vi "ShowWindow Wrapper Template.vi"(0 "hWnd":u64, 5 "nCmdShow":i32=4, 11 "error in":errorcluster) -> (4 "return value":i32, 15 "error out":errorcluster)   [LabVIEW 2020]
doc: "Sets the show state of the window hWnd through user32.dll ShowWindow (stdcall, called in any thread). nCmdShow 4 SW_SHOWNOACTIVATE restores a minimized window without activating it; 9 SW_RESTORE restores and activates; 0 SW_HIDE hides it. When error in carries an error the DLL is not called. Generated by tools\\Build Win32 Wrappers.vi - do not edit by hand, rebuild it."
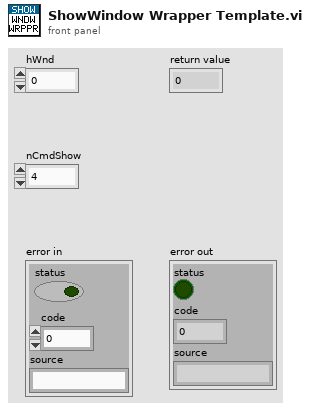
[diagram p1: front panel]
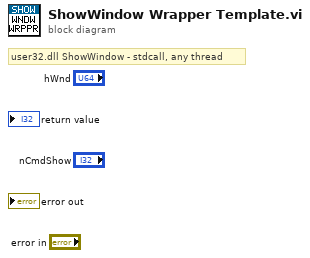
[diagram p0: block diagram]
diagram:
  # "user32.dll ShowWindow - stdcall, any thread"
